vi "Read Parameters.vi"(8 "error in (no error)":errorcluster, 11 "Selec Refn":T6) -> (0 "error out":errorcluster, 3 "Selec":T1={"1Dig"=enum."Black - 0", "2Dig"=enum."Black - 0", "3Dig"=enum."Black - 0", "Mul"=enum."Silver - x 0.01", "Tol"=enum."Gold - 5%", "TC"=enum."Grey - 1 ppm/K"})   [LabVIEW 2018]
doc: "Reads the selected values from the resistor band Enum controls on the Front Panel.\n\nThe VI receives the <b>Selec Refn</b> cluster containing the references to the six Enum controls and reads their current values.\n\nThe selected values are grouped into the <b>Selec</b> cluster, which contains the parameters for the first, second, and third significant digits, multiplier, tolerance, and temperature coefficient.\n\nThe VI propagates errors through its <b>error in</b> and <b>error out</b> terminals."
uses:
  Resistor Controls/Selectors Refnums--cluster.ctl
  Resistor Controls/Digit--enum.ctl
  Resistor Controls/Multiplier--enum.ctl
  Resistor Controls/Tolerance--enum.ctl
  Resistor Controls/Temp Coefficient--enum.ctl
  Resistor Controls/Selectors--cluster.ctl
  Resistor Controls/Resistance Controls.lvlib
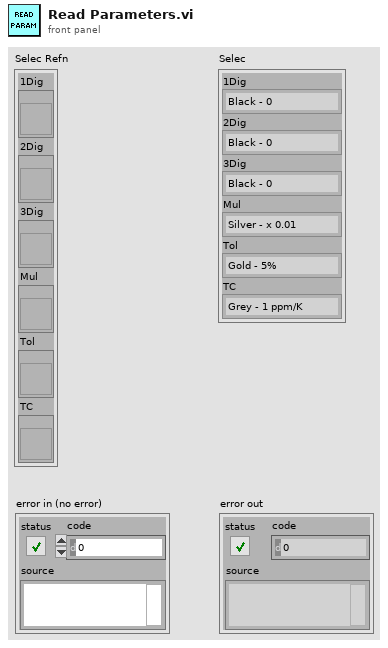
[diagram p1: front panel]
types:
  T1 = typedef "Resistance Controls.lvlib/Selectors--cluster.ctl" = cluster{"1Dig":T2, "2Dig":T2, "3Dig":T2, "Mul":T3, "Tol":T4, "TC":T5}
  T2 = typedef "Resistance Controls.lvlib/Digit--enum.ctl" = enum16{"Black - 0", "Brown - 1", "Red - 2", "Orange - 3", "Yellow - 4", "Green - 5", "Blue - 6", "Violet - 7", "Grey - 8", "White - 9"}
  T3 = typedef "Resistance Controls.lvlib/Multiplier--enum.ctl" = enum16{"Silver - x 0.01", "Gold - x 0.1 ", "Black - x 1", "Brown - x 10", "Red - x 100", "Orange - x 1k", "Yellow - x 10k", "Green - 100k", "Blue - x 1M", "Violet - x10 M", "Grey - x 100M", "White - x 1G"}
  T4 = typedef "Resistance Controls.lvlib/Tolerance--enum.ctl" = enum16{"Gray - 0.05%", "Violet - 0.1%", "Blue - 0.25%", "Green - 0.5%", "Brown - 1%", "Red - 2%", "Gold - 5%", "Silver - 10%", "None - 20%"}
  T5 = typedef "Resistance Controls.lvlib/Temp Coefficient--enum.ctl" = enum16{"Grey - 1 ppm/K", "Violet - 5 ppm/K", "Blue - 10 ppm/K", "Green - 20 ppm/K", "Yellow - 25 ppm/K", "Orange - 15 ppm/K", "Red - 50 ppm/K", "Brown - 100 ppm/K", "Black - 250 ppm/K"}
  T6 = typedef "Resistance Controls.lvlib/Selectors Refnums--cluster.ctl" = cluster{"1Dig":refnum<vi>, "2Dig":refnum<vi>, "3Dig":refnum<vi>, "Mul":refnum<vi>, "Tol":refnum<vi>, "TC":refnum<vi>}
  T7 = typedef "digit--enum.ctl" = enum16{"Black - 0", "Brown - 1", "Red - 2", "Orange - 3", "Yellow - 4", "Green - 5", "Blue - 6", "Violet - 7", "Grey - 8", "White - 9"}
  T8 = typedef "multiplier--enum.ctl" = enum16{"Silver - x 0.01", "Gold - x 0.1 ", "Black - x 1", "Brown - x 10", "Red - x 100", "Orange - x 1k", "Yellow - x 10k", "Green - 100k", "Blue - x 1M", "Violet - x10 M", "Grey - x 100M", "White - x 1G"}
  T9 = typedef "tolerance--enum.ctl" = enum16{"Gray - 0.05%", "Violet - 0.1%", "Blue - 0.25%", "Green - 0.5%", "Brown - 1%", "Red - 2%", "Gold - 5%", "Silver - 10%", "None - 20%"}
  T10 = typedef "temp coeficient--enum.ctl" = enum16{"Grey - 1 ppm/K", "Violet - 5 ppm/K", "Blue - 10 ppm/K", "Green - 20 ppm/K", "Yellow - 25 ppm/K", "Orange - 15 ppm/K", "Red - 50 ppm/K", "Brown - 100 ppm/K", "Black - 250 ppm/K"}
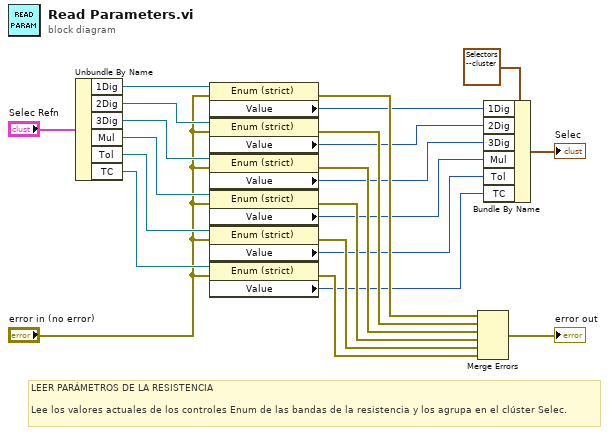
[diagram p0: block diagram]
diagram:
  # "LEER PARÁMETROS DE LA RESISTENCIA\n\nLee los valores actuales de los controles Enum de las bandas de la resistencia y los agrupa en el clúster Selec."
  n1 = Unbundle By Name("Selec Refn") -> ("1Dig"=w16:refnum<vi>, "2Dig"=w15:refnum<vi>, "3Dig"=w14:refnum<vi>, "Mul"=w13:refnum<vi>, "Tol"=w12:refnum<vi>, "TC"=w11:refnum<vi>)
  n2 = property class="Enum (strict)"(reference=w16, error in="error in (no error)") -> (error out=w23:errorcluster, "Value"=w10:T7)  [unwired: 1 out]
  n3 = property class="Enum (strict)"(reference=w15, error in="error in (no error)") -> (error out=w22:errorcluster, "Value"=w9:T7)  [unwired: 1 out]
  n4 = property class="Enum (strict)"(reference=w14, error in="error in (no error)") -> (error out=w21:errorcluster, "Value"=w8:T7)  [unwired: 1 out]
  n5 = property class="Enum (strict)"(reference=w13, error in="error in (no error)") -> (error out=w20:errorcluster, "Value"=w7:T8)  [unwired: 1 out]
  n6 = property class="Enum (strict)"(reference=w12, error in="error in (no error)") -> (error out=w19:errorcluster, "Value"=w6:T9)  [unwired: 1 out]
  n7 = property class="Enum (strict)"(reference=w11, error in="error in (no error)") -> (error out=w18:errorcluster, "Value"=w5:T10)  [unwired: 1 out]
  n8 = Merge Errors(w23, w22, w21, w20, w19, w18) -> (→"error out":errorcluster)
  n9 = Bundle By Name(cluster=T1 {"1Dig"=enum."Black - 0", "2Dig"=enum."Black - 0", "3Dig"=enum."Black - 0", "Mul"=enum."Silver - x 0.01", "Tol"=enum."Gold - 5%", "TC"=enum."Grey - 1 ppm/K"} ("Selec"), "1Dig"=w10, "2Dig"=w9, "3Dig"=w8, "Mul"=w7, "Tol"=w6, "TC"=w5) -> (→"Selec":T1)
